vi "Data handler-Acquisition protocols.vi"(0 "Data-gen queue":T6, 1 "Image array":T2, 2 "UI queue":refnum<queue>, 3 "Live graph data queue in":T4, 4 "Channel info":T1, 5 "Number of files closed in in":u32, 7 "Enable ref saving":bool, 9 "Logging queue element in":T7={"Imaging Protocol"=enum."Live Imaging", "Number of Trials"=0, "Frame Size"=512, "# Averaged frames"=0, "Dwell time (us)"=0.0, "Index of Z-plane"=0, "Timelapse?"=FALSE, "Logging process is active"=FALSE, "Speed logging enabled"=FALSE, "tdms file ref"=refnum, "path"=path "", "Trial Number"=0, "Expected # points acquired"=FALSE, "Manually stopped"=FALSE, "Last trial"=FALSE, "Ch0 data"=[], "Ch1 data"=[], "Ref Data"=[], "Ref Frame Time"=[], "Image Time"=[], "Continuous Time"=[], "Ref X Length"=0, "Ref Y Length"=0, "# Ref Averaged frames"=0, "Ref Dwell time (us)"=0.0, "Points acquired"={"Ch0 last trial"=0, "Ch1 last trial"=0, "All trials"=0}, "HW Timings File"=refnum} {"Ref Dwell time (us)" format="%#.6g"; "Frame Size" items=["100X100"=100, "128X128"=128, "200X200"=200, "256X256"=256, "512X512"=512, "1024x1024"=1024, "2048x2048"=2048]; "Dwell time (us)" format="%#.6g"}, 11 "Single Frame Data":T5, 12 "Movement Correction":bool, 14 "Save Reference":bool) -> (6 "Number of files closed out":u32, 15 "error out":errorcluster)   [LabVIEW 2020]
uses:
  Typedefs/Logging queue element.ctl
  Typedefs/Imaging Protocols enum.ctl
  Typedefs/Frame Size.ctl
  Typedefs/Acquired points count.ctl
  Typedefs/ROI File Generator Queue Ref.ctl
  Typedefs/Frame data dual cluster.ctl
  User Interface/Typedefs/Live graph data queue ref.ctl
  User Interface/Queue/Live graphs queue/Typedefs/Live imaging queue element.ctl
  <vilib>/vision/Image Controls.llb/IMAQ Image.ctl
  User Interface/Queue/Message Queue/Typedefs/Message Cluster.ctl
  Typedefs/Start-Stop Enum.ctl
  Typedefs/Channel Selector.ctl
  Global Variables/General Globals.vi
panel:
  out "Last trial?":bool
  out "Expected # points acquired":bool
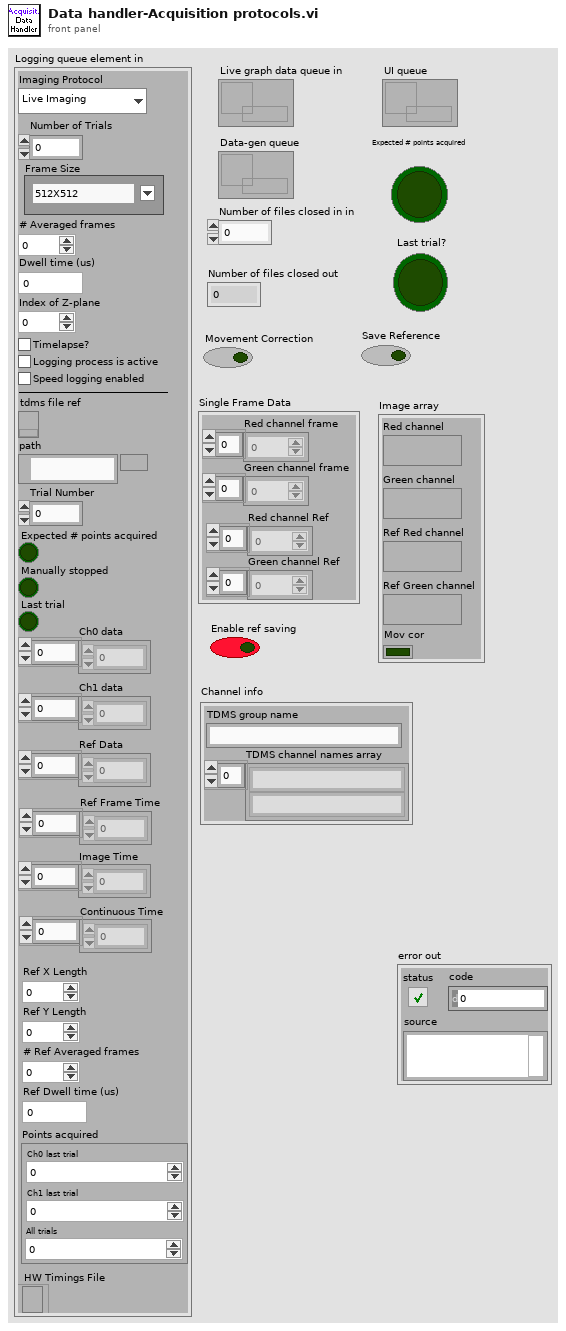
[diagram p1: front panel]
types:
  T1 = cluster{"TDMS group name":string, "TDMS channel names array":string[]}
  T2 = typedef "Live imaging queue element.ctl" = cluster{"Red channel":T3, "Green channel":T3, "Ref Red channel":T3, "Ref Green channel":T3, "Mov cor":bool}
  T3 = typedef "IMAQ Image.ctl" = refnum<image>
  T4 = typedef "Live graph data queue ref.ctl" = refnum<queue>
  T5 = typedef "Frame data dual cluster.ctl" = cluster{"Red channel frame":dbl[], "Green channel frame":dbl[], "Red channel Ref":dbl[], "Green channel Ref":dbl[]}
  T6 = typedef "ROI File Generator Queue Ref.ctl" = refnum<queue>
  T7 = typedef "Logging queue element.ctl" = cluster{"Imaging Protocol":T8, "Number of Trials":u16, "Frame Size":T9, "# Averaged frames":u16, "Dwell time (us)":dbl, "Index of Z-plane":i32, "Timelapse?":bool, "Logging process is active":bool, "Speed logging enabled":bool, "tdms file ref":refnum<k34>, "path":path, "Trial Number":i32, "Expected # points acquired":bool, "Manually stopped":bool, "Last trial":bool, "Ch0 data":u32[], "Ch1 data":u32[], "Ref Data":u32[], "Ref Frame Time":u64[], "Image Time":u64[], "Continuous Time":u64[], "Ref X Length":u16, "Ref Y Length":u16, "# Ref Averaged frames":u16, "Ref Dwell time (us)":dbl, "Points acquired":T10, "HW Timings File":refnum<file>}
  T8 = typedef "Imaging Protocols enum.ctl" = enum16{"AOL Z-Stack", "Motor Z Stack", "Functional Acquisition", "Single Plane Acquisition", "Volume Acquisition", "Live Imaging", "Live Plane Imaging", "Live Volume Imaging"}
  T9 = typedef "Frame Size.ctl" = u16
  T10 = typedef "Acquired points count.ctl" = cluster{"Ch0 last trial":u64, "Ch1 last trial":u64, "All trials":u64}
  T11 = typedef "Start-Stop Enum.ctl" = enum16{"START", "STOP"}
  T12 = typedef "Channel Selector.ctl" = enum16{"Red Channel", "Green Channel", "Blended"}
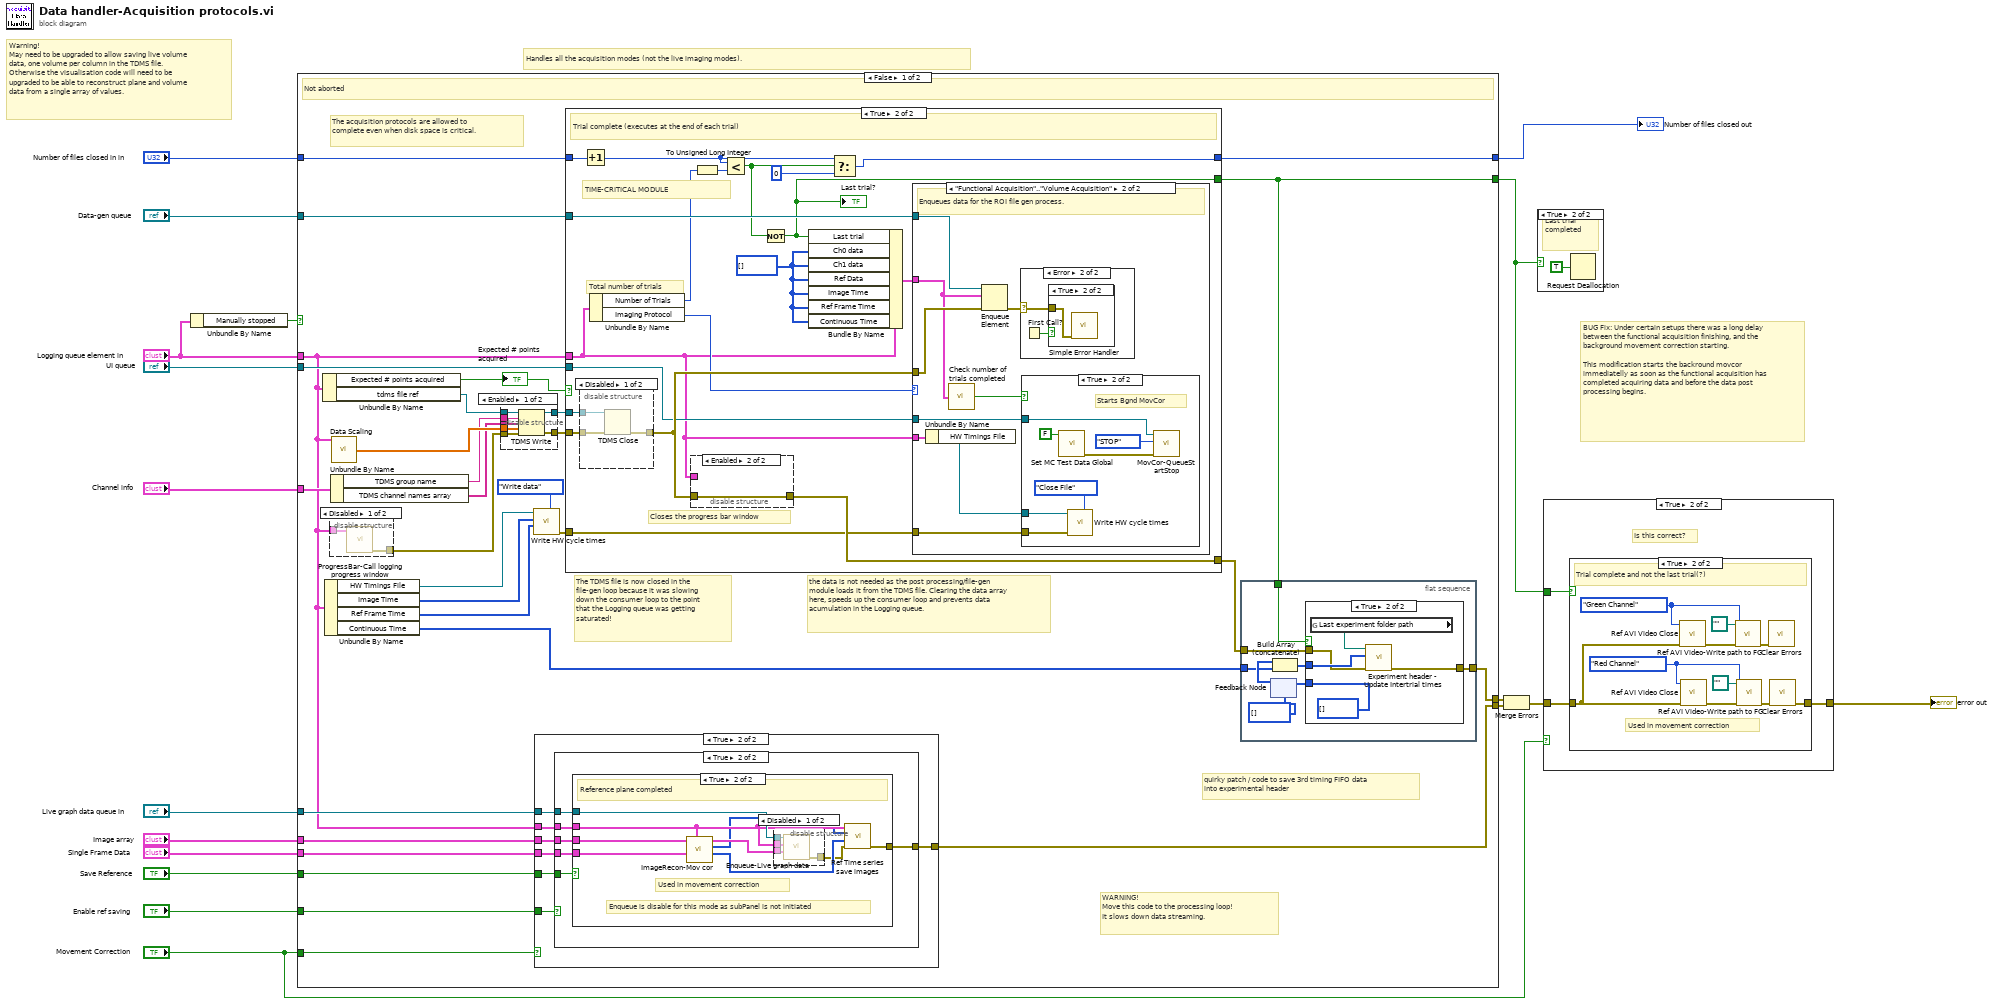
[diagram p0: block diagram]
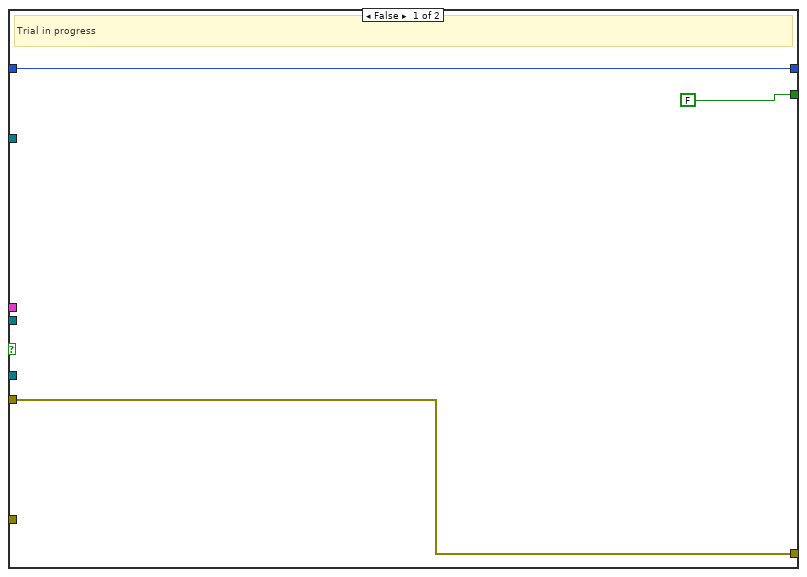
[diagram p6: hidden frame]
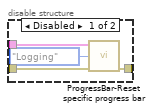
[diagram p11: hidden frame]
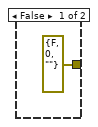
[diagram p13: hidden frame]
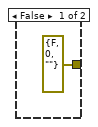
[diagram p14: hidden frame]
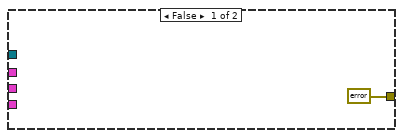
[diagram p15: hidden frame]
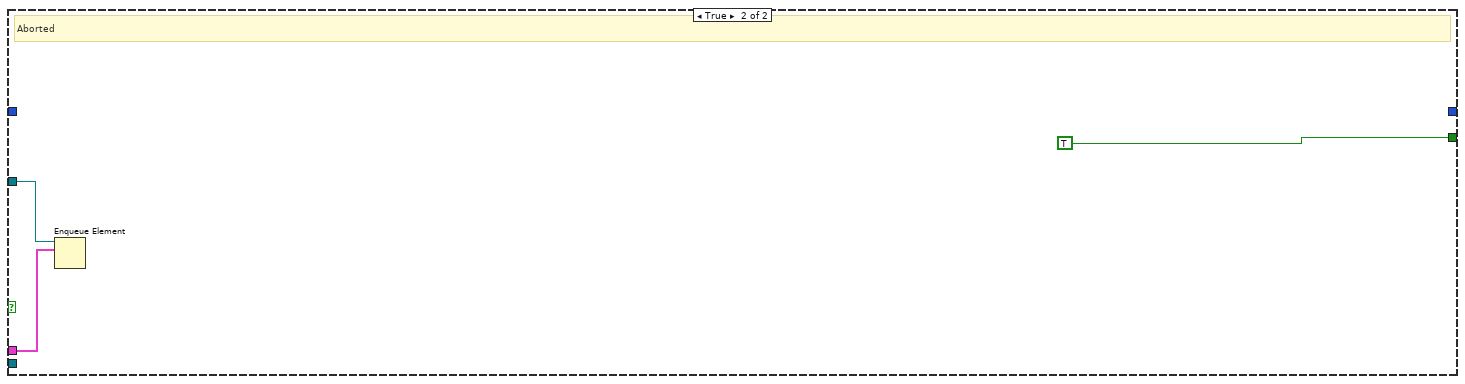
[diagram p17: hidden frame]
diagram:
  # "Warning!\nMay need to be upgraded to allow saving live volume data, one volume per column in the TDMS file. Otherwise the visualisation code will need to be upgraded to be able to reconstruct plane and volume data from a single array of values."
  # "Handles all the acquisition modes (not the live imaging modes)."
  # "BUG Fix: Under certain setups there was a long delay between the functional acquisition finishing, and the background movement correction starting.\n\nThis modification starts the backround movcor immediatelly as soon as the functional acquisition has completed acquiring data and before the data post processing begins."
  n1 = Unbundle By Name("Logging queue element in") -> ("Manually stopped"=w2:bool)
  n2 = case shown="False" w2 {
    tunnel: "Data-gen queue" -> [w48 w153]
    tunnel: [w47 _] -> w17
    tunnel: "Number of files closed in in" -> [w46 _]
    tunnel: "Live graph data queue in" -> [w40 _]
    tunnel: "Logging queue element in" -> [w28 w152]
    tunnel: "Single Frame Data" -> [w39 _]
    tunnel: "Image array" -> [w38 _]
    tunnel: "Save Reference" -> [w37 _]
    tunnel: [w36 _] -> w10
    tunnel: [w19 _] -> w9
    tunnel: "Enable ref saving" -> [w35 _]
    tunnel: "Movement Correction" -> [w34 _]
    tunnel: [w20 TRUE] -> w7
    tunnel: "Channel info" -> [w32 _]
    tunnel: "UI queue" -> [w29 _]
    frame False {
      # "quirky patch / code to save 3rd timing FIFO data \ninto experimental header"
      # "WARNING!\nMove this code to the processing loop!\nIt slows down data streaming."
      # "The TDMS file is now closed in the file-gen loop because it was slowing down the consumer loop to the point that the Logging queue was getting saturated!"
      # "the data is not needed as the post processing/file-gen module loads it from the TDMS file. Clearing the data array here, speeds up the consumer loop and prevents data acumulation in the Logging queue."
      # "The acquisition protocols are allowed to complete even when disk space is critical."
      # "Not aborted"
      n3 = Unbundle By Name(w28) -> ("Expected # points acquired"=w42:bool, "tdms file ref"=w43:refnum<k34>)
      "Expected # points acquired" <- w42
      n4 = Unbundle By Name(w28) -> ("HW Timings File"=w24:refnum<file>, "Image Time"=w26:u64[], "Ref Frame Time"=w25:u64[], "Continuous Time"=w22:u64[])
      n5 = disable-structure shown="Disabled" {
        disable-tunnel: [w72 _] -> w41
        disable-tunnel: w28 -> [w71 _]
        frame Disabled {
          n6 = call "ProgressBar-Call logging progress window.vi"("Z-stack queue cluster"=w71) -> ("error out"=w72:errorcluster)  [unwired: 10 in]
        }
        frame Enabled {
        }
      }
      n7 = Unbundle By Name(w32) -> ("TDMS group name"=w31:string, "TDMS channel names array"=w30:string[])
      n8 = call "Data Scaling.vi"("Logging queue element in"=w28) -> ("Two channel data"=w33:dbl[][])  [unwired: 13 in, 1 out]
      n9 = disable-structure shown="Enabled" {
        disable-tunnel: [w70 _] -> w45
        disable-tunnel: [w69 _] -> w44
        disable-tunnel: w43 -> [w68 _]
        disable-tunnel: w30 -> [w67 _]
        disable-tunnel: w31 -> [w66 _]
        disable-tunnel: w41 -> [w65 _]
        disable-tunnel: w33 -> [w64 _]
        frame Enabled {
          n10 = TDMS Write(0:w68, 5:w66, 7:w67, 9:w64, 11:w65) -> (4:w69:refnum<k34>, 15:w70:errorcluster)  [unwired: 1 in, 2 out]
        }
        frame Disabled {
        }
      }
      n11 = call "Write HW cycle times.vi"("Function"=enum16{"Open file", "Write data", "Close File"}."Write data", "Ref Time Stamps in"=w25, "Image Time in"=w26, "HW Timings File"=w24) -> ("error out"=w23:errorcluster)  [unwired: 6 in, 1 out]
      n12 = case shown="True" w34 {
        tunnel: w40 -> [_ w130]
        tunnel: w28 -> [_ w129]
        tunnel: w39 -> [_ w128]
        tunnel: w38 -> [_ w127]
        tunnel: w37 -> [_ w126]
        tunnel: [errorcluster {"status"=FALSE, "code"=0, "source"=""} ("error") w125] -> w36
        tunnel: w35 -> [_ w124]
        frame False {
        }
        frame True {
          n13 = case shown="True" w124 {
            tunnel: w130 -> [_ w137]
            tunnel: w129 -> [_ w136]
            tunnel: w128 -> [_ w135]
            tunnel: w127 -> [_ w134]
            tunnel: w126 -> [_ w133]
            tunnel: [errorcluster {"status"=FALSE, "code"=0, "source"=""} ("error") w132] -> w125
            frame False {
            }
            frame True {
              n14 = case shown="True" w133 {
                tunnel: w136 -> [_ w144]
                tunnel: [errorcluster {"status"=FALSE, "code"=0, "source"=""} ("error out") w147] -> w132
                tunnel: w137 -> [_ w146]
                tunnel: w134 -> [_ w145]
                tunnel: w135 -> [_ w142]
                frame False {
                }
                frame True {
                  # "Enqueue is disable for this mode as subPanel is not initiated"
                  # "Used in movement correction"
                  # "Reference plane completed"
                  n15 = call "ImageRecon-Mov cor.vi"("Logging queue element in"=w144, "Data"=w142, "Image Array (in)"=w145) -> ("Ch1-Green-REF"=w140:i16[][], "Ch0-Red-REF"=w141:i16[][], "Image Array(out)"=w143:T2)  [unwired: 5 in, 1 out]
                  n16 = disable-structure shown="Disabled" {
                    disable-tunnel: w146 -> [w151 _]
                    disable-tunnel: w144 -> [w150 _]
                    disable-tunnel: w143 -> [w149 _]
                    disable-tunnel: [w148 _] -> w139
                    frame Disabled {
                      n17 = call "Enqueue-Live graph data.vi"("Element to queue"=w149, "Logging queue element"=w150, "Live graph data queue in"=w151) -> ("error out"=w148:errorcluster)  [unwired: 7 in, 1 out]
                    }
                    frame Enabled {
                    }
                  }
                  n18 = call "Ref Time series save images.vi"("error in (no error)"=w139, "Ch1-Green-REF"=w140, "Ch0-Red-REF"=w141, "Logging queue element"=w144) -> ("error"=w147:errorcluster)  [unwired: 7 in]
                }
              }
            }
          }
        }
      }
      n19 = case shown="True" w42 {
        tunnel: w45 -> [w75 w94]
        tunnel: w44 -> [_ w93]
        tunnel: [w75 w79] -> w21
        tunnel: w48 -> [_ w92]
        tunnel: w28 -> [_ w77]
        tunnel: [w74 w88] -> w47
        tunnel: w46 -> [w74 w91]
        tunnel: [FALSE w82] -> w20
        tunnel: w29 -> [_ w80]
        tunnel: w23 -> [_ w78]
        frame False {
          # "Trial in progress"
        }
        frame True {
          w76 = u32[] [] ("Raw Data")
          # "TIME-CRITICAL MODULE"
          # "Total number of trials"
          # "Closes the progress bar window"
          # "Trial complete (executes at the end of each trial)"
          n20 = disable-structure shown="Disabled" {
            disable-tunnel: w94 -> [w121 w122]
            disable-tunnel: w93 -> [w120 _]
            disable-tunnel: [w119 w122] -> w90
            frame Disabled {
              n21 = TDMS Close(8:w121, 11:w120) -> (0:w119:errorcluster)  [unwired: 1 out]
            }
            frame Enabled {
            }
          }
          n22 = Increment(x=w91) -> (x+1=w83:u32)
          n23 = Unbundle By Name(w77) -> ("Number of Trials"=w89:u16, "Imaging Protocol"=w81:T8)
          n24 = disable-structure shown="Enabled" {
            disable-tunnel: [w116 w118] -> w79
            disable-tunnel: w90 -> [w115 w118]
            disable-tunnel: w77 -> [w114 _]
            frame Disabled {
              n25 = call "ProgressBar-Reset specific progress bar.vi"("Error in"=w115, "Sender"=enum16{"Acquisition", "Logging", "File gen"}."Logging", "Z-stack queue cluster"=w114) -> ("error out"=w116:errorcluster)  [unwired: 8 in]
            }
            frame Enabled {
            }
          }
          n26 = To Unsigned Long Integer(number=w89) -> (unsigned 32bit integer=w86:u32)
          n27 = Less?(x=w83, y=w86) -> (x < y?=w85:bool)
          n28 = Not(x=w85) -> (.not. x?=w82:bool)
          "Last trial?" <- w82
          n29 = Bundle By Name(cluster=w77, "Last trial"=w82, "Ch0 data"=w76, "Ch1 data"=w76, "Ref Data"=w76, "Image Time"=w76, "Ref Frame Time"=w76, "Continuous Time"=w76) -> (w84:T7)
          n30 = Select(t=w83, s=w85, f=u32 0) -> (s? t:f=w88:u32)
          n31 = case shown="\"Functional Acquisition\"..\"Volume Acquisition\"" w81 {
            tunnel: w90 -> [_ w101]
            tunnel: w92 -> [_ w103]
            tunnel: w84 -> [_ w100]
            tunnel: w80 -> [_ w98]
            tunnel: w78 -> [_ w97]
            tunnel: w77 -> [_ w96]
            frame Default {
              # "Unhandled modes"
            }
            frame "Functional Acquisition".."Volume Acquisition" {
              # "Enqueues data for the ROI file gen process."
              n32 = Unbundle By Name(w96) -> ("HW Timings File"=w95:refnum<file>)
              n33 = call "Check number of trials completed.vi"("Cluster"=w100) -> ("# of trials completed"=w99:bool)
              n34 = Enqueue Element(queue=w103, element=w100, error in (no error)=w101) -> (error out=w102:errorcluster)  [unwired: 1 in, 2 out]
              n35 = case shown="Error" w102 {
                selector: w102 -> [_ w112]
                frame No Error {
                }
                frame Error {
                  n36 = First Call?() -> (First Call?: T/F=w111:bool)
                  n37 = case shown="True" w111 {
                    tunnel: w112 -> [_ w113]
                    frame False {
                    }
                    frame True {
                      n38 = call <vilib>:"Simple Error Handler.vi"("error in (no error)"=w113) -> ()  [unwired: 4 in, 5 out]
                    }
                  }
                }
              }
              n39 = case shown="True" w99 {
                tunnel: w98 -> [_ w107]
                tunnel: w97 -> [_ w105]
                tunnel: w95 -> [_ w104]
                frame False {
                }
                frame True {
                  # "Starts Bgnd MovCor"
                  n40 = call "Set MC Test Data Global.vi"("Save MC TestData"=FALSE) -> ("error out"=w110:errorcluster)  [unwired: 9 in, 1 out]
                  n41 = call "Write HW cycle times.vi"("Function"=enum16{"Open file", "Write data", "Close File"}."Close File", "error in (no error)"=w105, "HW Timings File"=w104) -> ()  [unwired: 7 in, 2 out]
                  n42 = call "MovCor-QueueStartStop.vi"("error in (no error)"=w110, "Main prrotocol Starting/Stopped"=Start-Stop_Enum."STOP" ("Start/Stop"), "UI queue in"=w107) -> ()  [unwired: 7 in, 2 out]
                }
              }
            }
          }
        }
      }
      n43 = flat-sequence {
        tunnel: w22 -> [w55]
        tunnel: w21 -> [w50]
        tunnel: w20 -> [w53]
        tunnel: [w49] -> w19
        frame #0 {
          n44 = feedback #1(u64[] []) -> (w56:u64[])
          n45 = Build Array (concatenate)(w56, w55) -> (w52:u64[])
          n46 = case shown="True" w53 {
            tunnel: w52 -> [w58 w61]
            tunnel: [w58 u64[] []] -> w51
            tunnel: w50 -> [w57 w60]
            tunnel: [w57 w59] -> w49
            frame False {
            }
            frame True {
              n47 = global read "General Globals.vi" "Last experiment folder path"() -> (w62:path)
              n48 = call "Experiment header - Update Intertrial times.vi"("error in"=w60, "Array"=w61, "Experiment folder path"=w62) -> ("error out"=w59:errorcluster)  [unwired: 8 in]
            }
          }
          n49 = feedback-in #1(w51) -> ()
        }
      }
    }
    frame True {
      # "Aborted"
      n50 = Enqueue Element(queue=w153, element=w152) -> ()  [unwired: 2 in, 3 out]
    }
  }
  "Number of files closed out" <- w17
  n51 = Merge Errors(w9, w10) -> (w11:errorcluster)
  n52 = case shown="True" w7 {
    frame False {
    }
    frame True {
      # "Last trial completed"
      n53 = Request Deallocation(TRUE ("flag")) -> ()
    }
  }
  n54 = case shown="True" "Movement Correction" {
    tunnel: w11 -> [w156 w159]
    tunnel: w7 -> [_ w158]
    tunnel: [w156 w157] -> w4
    frame False {
    }
    frame True {
      # "Is this correct?"
      n55 = case shown="True" w158 {
        tunnel: w159 -> [w160 w164]
        tunnel: [w160 w161] -> w157
        frame False {
        }
        frame True {
          w162 = Channel_Selector."Red Channel" ("Channel")
          w163 = Channel_Selector."Green Channel" ("Channel")
          # "Used in movement correction"
          # "Trial complete and not the last trial(?)"
          n56 = call "Ref AVI Video Close.vi"("error in (no error)"=w164, "Channel"=w163) -> ("error out"=w170:errorcluster)  [unwired: 9 in]
          n57 = call "Ref AVI Video Close.vi"("error in (no error)"=w164, "Channel"=w162) -> ("error out"=w165:errorcluster)  [unwired: 9 in]
          n58 = call "Ref AVI Video-Write path to FG.vi"("error in (no error)"=w170, "Channel"=w163, "AVI2 path"=path "") -> ("error out"=w168:errorcluster)  [unwired: 8 in]
          n59 = call "Ref AVI Video-Write path to FG.vi"("error in (no error)"=w165, "Channel"=w162, "AVI2 path"=path "") -> ("error out"=w167:errorcluster)  [unwired: 8 in]
          n60 = call <vilib>:"Clear Errors.vi"("error in (no error)"=w168) -> ()  [unwired: 5 in, 2 out]
          n61 = call <vilib>:"Clear Errors.vi"("error in (no error)"=w167) -> ("error out"=w161:errorcluster)  [unwired: 5 in, 1 out]
        }
      }
    }
  }
  "error out" <- w4
